vi "Is Reentrant Measurement.vi"(8 "error in (no error)":errorcluster, 11 "measurement plugin service in":refnum<class "Measurement Plugin Service.lvclass">) -> (0 "error out":errorcluster, 1 "is reentrant":bool, 3 "measurement plugin service out":refnum<class "Measurement Plugin Service.lvclass">)   [LabVIEW 2021, in "NI Measurement Plug-In SDK.lvlib" / "Measurement Plugin Service.lvclass"]
uses:
  Measurement Plugin Service.lvclass
  Measurement Plugin Service.lvclass/Measurement Plugin Service.ctl
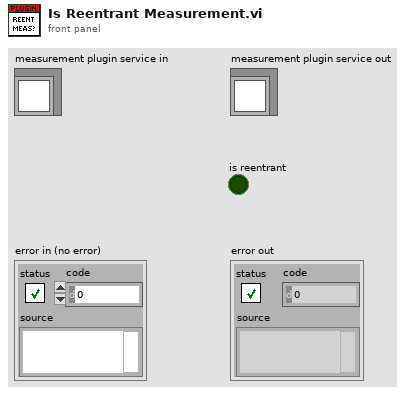
[diagram p1: front panel]
types:
  T1 = typedef "NI Measurement Plug-In SDK.lvlib/Measurement Plugin Service.lvclass/Plugin Paths.ctl" = cluster{"get service descriptor VI path":path, "get type specializations VI path":path, "get UI details VI path":path, "measurement logic VI path":path, "measurement configuration ctl path":path, "measurement results ctl path":path}
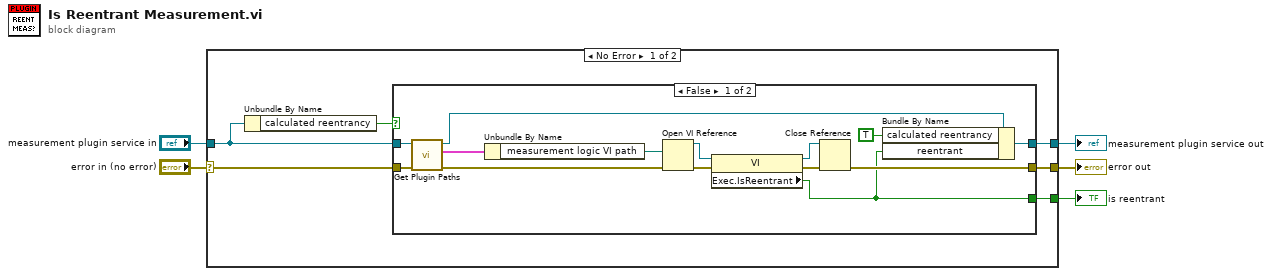
[diagram p0: block diagram]
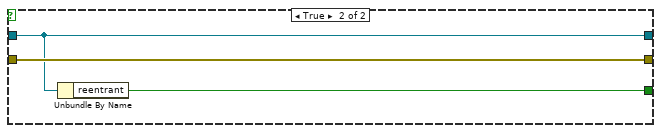
[diagram p2: hidden frame]
diagram:
  n1 = case shown="No Error" "error in (no error)" {
    selector: "error in (no error)" -> [w10 w30]
    tunnel: [w8 w30] -> w4
    tunnel: [w9 w29] -> w2
    tunnel: "measurement plugin service in" -> [w11 w29]
    tunnel: [w7 _] -> w1
    frame No Error {
      n2 = Unbundle By Name(w11) -> ("calculated reentrancy"=w6:bool)
      n3 = case shown="False" w6 {
        tunnel: w11 -> [w25 w27]
        tunnel: w10 -> [w24 w28]
        tunnel: [w14 w27] -> w9
        tunnel: [w15 w28] -> w8
        tunnel: [w13 w26] -> w7
        frame False {
          n4 = call-dynamic "Get Plugin Paths.vi"("error in"=w24, "measurement plugin service in"=w25) -> ("error out"=w20:errorcluster, "plugin paths"=w23:T1, "measurement plugin service out"=w22:refnum<class "Measurement Plugin Service.lvclass">)  [unwired: 7 in]
          n5 = Unbundle By Name(w23) -> ("measurement logic VI path"=w21:path)
          n6 = Open VI Reference(vi path=w21, error in (no error)=w20) -> (vi reference=w19:refnum<vi>, error out=w18:errorcluster)  [unwired: 4 in]
          n7 = property class="VI"(reference=w19, error in=w18) -> (reference out=w16:refnum<vi>, error out=w17:errorcluster, "Exec.IsReentrant"=w13:bool)
          n8 = Close Reference(reference=w16, error in (no error)=w17) -> (error out=w15:errorcluster)
          n9 = Bundle By Name(cluster=w22, "calculated reentrancy"=TRUE, "reentrant"=w13) -> (w14:refnum<class "Measurement Plugin Service.lvclass">)
        }
        frame True {
          n10 = Unbundle By Name(w27) -> ("reentrant"=w26:bool)
        }
      }
    }
    frame Error {
    }
  }
  "error out" <- w4
  "measurement plugin service out" <- w2
  "is reentrant" <- w1
